vi "P7_RemoveBadWires.vi"(11 "Inputs":string[](array[string])) -> (2 "Output/Failure":string, 3 "CLI Process Return Code":i32)   [LabVIEW 2026]
doc: "Slice 1.1 probe: Open VI Reference on a VI with one broken wire, read Wires[] and Is Broken?, BD.Remove Bad Wires, read Wires[] again, close the reference."
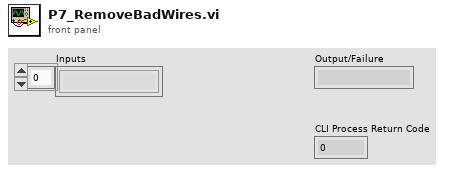
[diagram p1: front panel]
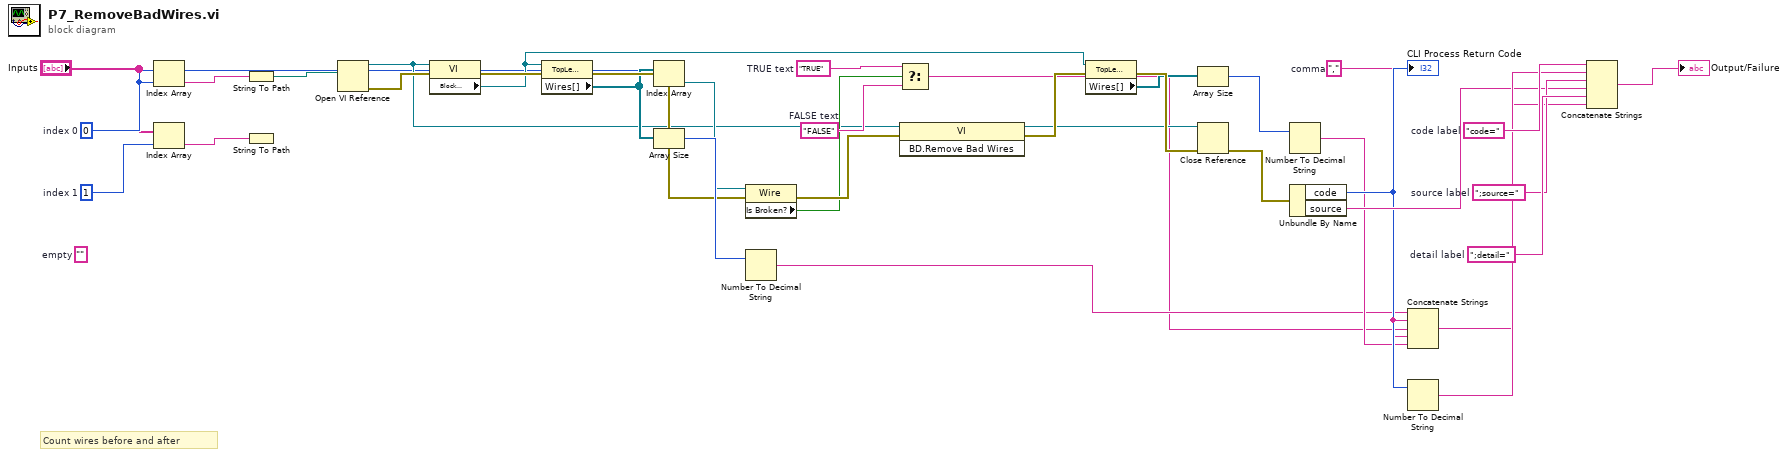
[diagram p0: block diagram]
diagram:
  w35 = ";detail="  # detail label
  w34 = ";source="  # source label
  w33 = "code="  # code label
  w23 = ","  # comma
  w17 = "FALSE"  # FALSE text
  w16 = "TRUE"  # TRUE text
  (unwired) ""  # empty
  w3 = 1  # index 1
  w2 = 0  # index 0
  # "Count wires before and after"
  n1 = Index Array(array="Inputs", index=w2) -> (element=w4:string)
  n2 = Index Array(array="Inputs", index=w3) -> (element=w5:string)
  n3 = String To Path(string=w4) -> (path=w6:path)
  n4 = String To Path(string=w5) -> ()  [unwired: 1 out]
  n5 = Open VI Reference(vi path=w6) -> (vi reference=w7:refnum<vi>, error out=w8:errorcluster)  [unwired: 5 in]
  n6 = property class="VI"(reference=w7, error in=w8) -> (error out=w10:errorcluster, "Block Diagram"=w9:refnum<vi>)  [unwired: 1 out]
  n7 = property class="TopLevelDiagram"(reference=w9, error in=w10) -> (error out=w12:errorcluster, "Wires[]"=w11:refnum<vi>[])  [unwired: 1 out]
  n8 = Index Array(array=w11, index=w2) -> (element=w13:refnum<vi>)
  n9 = Array Size(array=w11) -> (size(s)=w24:i32)
  n10 = property class="Wire"(reference=w13, error in=w12) -> (error out=w15:errorcluster, "Is Broken?"=w14:bool)  [unwired: 1 out]
  n11 = Number To Decimal String(number=w24) -> (decimal integer string=w25:string)  [unwired: 1 in]
  n12 = Select(t=w16, s=w14, f=w17) -> (s? t:f=w18:string)
  n13 = invoke class="VI" method="BD.Remove Bad Wires"(reference=w7, error in=w15) -> (reference out=w19:refnum<vi>, error out=w20:errorcluster)  [unwired: 1 in, 1 out]
  n14 = property class="TopLevelDiagram"(reference=w9, error in=w20) -> (error out=w22:errorcluster, "Wires[]"=w21:refnum<vi>[])  [unwired: 1 out]
  n15 = Array Size(array=w21) -> (size(s)=w26:i32)
  n16 = Close Reference(reference=w19, error in (no error)=w22) -> (error out=w29:errorcluster)
  n17 = Number To Decimal String(number=w26) -> (decimal integer string=w27:string)  [unwired: 1 in]
  n18 = Unbundle By Name(w29) -> ("code"=w30:i32, "source"=w31:string)
  "CLI Process Return Code" <- w30
  n19 = Concatenate Strings(w25, w23, w18, w23, w27) -> (w28:string)
  n20 = Number To Decimal String(number=w30) -> (decimal integer string=w32:string)  [unwired: 1 in]
  n21 = Concatenate Strings(w33, w32, w34, w31, w35, w28) -> (→"Output/Failure":string)
